vi "TDMS to Patch Image.vi"(0 "Experiment Path":path, 11 "error in (no error)":errorcluster, 12 "Imaging Protocol":T2=enum."Functional Acquisition", 13 "Predominant ROI type":T1=enum."Rectangle", 14 "No of Patches in Experiment":i32) -> (4 "Current Trial Number":i32, 6 "Cancelled":bool, 10 "All Files in Dir":path[](array[path]), 15 "error out":errorcluster)   [LabVIEW 2020]
uses:
  Globals/gl_funct TIFF export globals.vi
  Typedefs/Imaging Protocols enum.ctl
  Typedefs/ROI ID Enum.ctl
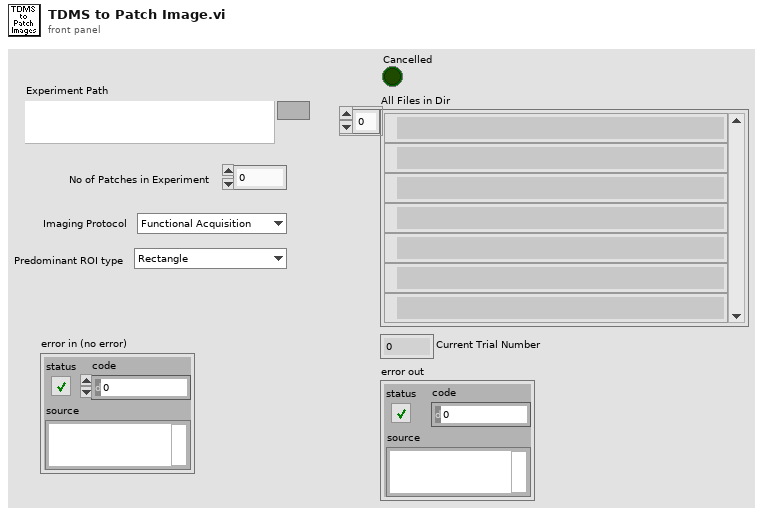
[diagram p1: front panel]
types:
  T1 = typedef "ROI ID Enum.ctl" = enum16{"Point", "MiniScan", "Comp. MiniScan", "Rectangle", "Comp. volume", "Arb. plane point", "None"}
  T2 = typedef "Imaging Protocols enum.ctl" = enum16{"AOL Z-Stack", "Motor Z Stack", "Parameter Sweep", "Functional Acquisition", "Single Plane Acquisition", "Volume Acquisition", "Live Imaging", "Live Plane Imaging", "Live Volume Imaging"}
  T3 = typedef "Funct TIFF exporter ctrl refs.ctl" = cluster{"This VI":refnum<vi>, "Current Experiment":refnum<vi>, "Imaging protocol":refnum<vi>, "Predominant ROI type":refnum<vi>, "Patches in Experiment":refnum<vi>, "Folder Path":refnum<vi>, "Export":refnum<vi>, "Trial number":refnum<vi>, "Output TIFF type":refnum<vi>}
  T4 = typedef "Exported TIFF type.ctl" = enum16{"One multi-page TIFF file for each rectangle", "Individual TIFF files"}
  T5 = typedef "Fixed strings.ctl" = cluster{"ROI file name":string, "Normalised ROI file name":string, "Zplane Pockels values file name":string, "Functional data folder name":string, "Experiment Header file name":string, "Z-stack images folder name":string, "Groups setup rel. path":string, "Groups text file rel. path":string, "TDMS files folder name (F.img)":string, "TDMS files folder name (V.acq)":string, "TDMS files folder name (Pl.acq)":string, "Cycle rel times sequence file":string, "Dynamically called VIs folder name":string, "Time Series folder base name":string, "Parameter Sweep":string}
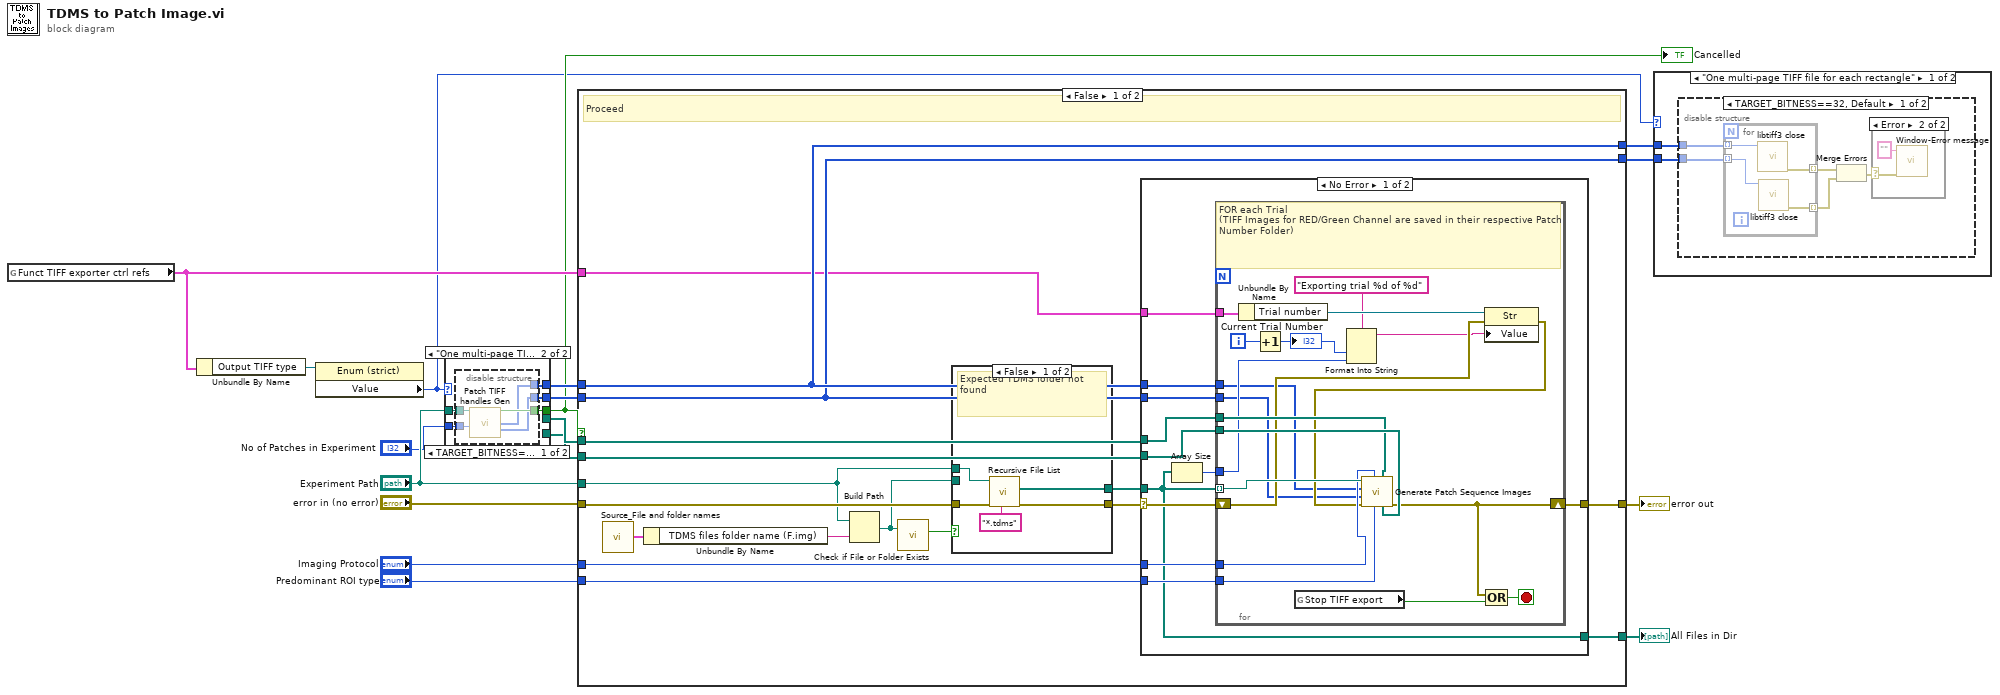
[diagram p0: block diagram]
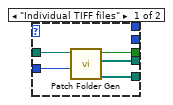
[diagram p5: hidden frame]
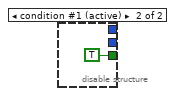
[diagram p6: hidden frame]
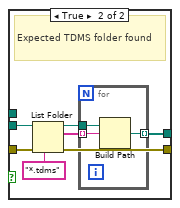
[diagram p7: hidden frame]
diagram:
  n1 = global read "gl_funct TIFF export globals.vi" "Funct TIFF exporter ctrl refs"() -> (w3:T3)
  n2 = Unbundle By Name(w3) -> ("Output TIFF type"=w4:refnum<vi>)
  n3 = property class="Enum (strict)"(reference=w4) -> ("Value"=w1:T4)  [unwired: 1 in, 2 out]
  n4 = case shown="\"One multi-page TIFF file for each rectangle\", Default" w1 {
    tunnel: [w22 _] -> w17
    tunnel: [w21 _] -> w16
    tunnel: [w20 w27] -> w2
    tunnel: "Experiment Path" -> [w19 w26]
    tunnel: "No of Patches in Experiment" -> [w18 w25]
    tunnel: [_ w24] -> w8
    tunnel: [_ w23] -> w7
    frame "Individual TIFF files" {
      n5 = call "Patch Folder Gen.vi"("No of Patches"=w18, "Experimental Folder"=w19) -> ("Green"=w21:path[], "Red"=w22:path[], "Cancelled"=w20:bool)  [unwired: 7 in]
    }
    frame "One multi-page TIFF file for each rectangle", Default {
      n6 = disable-structure shown="TARGET_BITNESS==32, Default" {
        disable-tunnel: [w32 TRUE ("Cancelled")] -> w27
        disable-tunnel: w26 -> [w31 _]
        disable-tunnel: w25 -> [w30 _]
        disable-tunnel: [w29 _] -> w24
        disable-tunnel: [w28 _] -> w23
        frame condition #0 {
          n7 = call "Patch TIFF handles Gen.vi"("Experimental Folder"=w31, "No of Patches"=w30) -> ("Cancelled"=w32:bool, "Red TIFF handles"=w29:i32[], "Green TIFF handles"=w28:i32[])  [unwired: 9 in, 2 out]
        }
        frame condition #1 (active) {
        }
      }
    }
  }
  "Cancelled" <- w2
  n8 = case shown="False" w2 {
    tunnel: w17 -> [w50 _]
    tunnel: w16 -> [w49 _]
    tunnel: "Imaging Protocol" -> [w48 _]
    tunnel: "Predominant ROI type" -> [w47 _]
    tunnel: [w46 w99] -> w12
    tunnel: "error in (no error)" -> [w44 w99]
    tunnel: [w45 _] -> w11
    tunnel: "Experiment Path" -> [w37 _]
    tunnel: w8 -> [w36 w98]
    tunnel: w7 -> [w35 w97]
    tunnel: [w36 w98] -> w6
    tunnel: [w35 w97] -> w5
    tunnel: w3 -> [w34 _]
    frame False {
      # "Proceed"
      n9 = call "Source_File and folder names.vi"() -> ("Fixed strings"=w41:T5)  [unwired: 1 in]
      n10 = Unbundle By Name(w41) -> ("TDMS files folder name (F.img)"=w40:string)
      n11 = Build Path(base path=w37, name or relative path=w40) -> (appended path=w38:path)
      n12 = call <vilib>:"Check if File or Folder Exists.vi"("path"=w38) -> ("file or folder exists?"=w39:bool)  [unwired: 8 in, 2 out]
      n13 = case shown="False" w39 {
        tunnel: w44 -> [w55 w62]
        tunnel: [w54 w61] -> w43
        tunnel: [w53 w56] -> w42
        tunnel: w38 -> [_ w60]
        tunnel: w37 -> [w51 _]
        frame False {
          # "Expected TDMS folder not found"
          n14 = call <vilib>:"Recursive File List.vi"("pattern"="*.tdms", "error in (no error)"=w55, "Folder Path"=w51) -> ("error out"=w54:errorcluster, "All Files in Dir"=w53:path[])  [unwired: 4 in, 3 out]
        }
        frame True {
          # "Expected TDMS folder found"
          n15 = List Folder(path=w60, pattern="*.tdms", error in=w62) -> (path out=w57:path, filenames=w58:string[], error out=w61:errorcluster)  [unwired: 1 in, 1 out]
          n16 = for {
            tunnel: w58 -> [w64] mode=indexing
            tunnel: w57 -> [w65]
            tunnel: [w63] -> w56 mode=indexing
            n17 = Build Path(base path=w65, name or relative path=w64) -> (appended path=w63:path)
          }
        }
      }
      n18 = case shown="No Error" w43 {
        selector: w43 -> [w71 w96]
        tunnel: w42 -> [w69 _]
        tunnel: w50 -> [w76 _]
        tunnel: w49 -> [w75 _]
        tunnel: w48 -> [w74 _]
        tunnel: w47 -> [w73 _]
        tunnel: [w72 w96] -> w46
        tunnel: [w69 _] -> w45
        tunnel: w34 -> [w70 _]
        tunnel: w36 -> [w67 _]
        tunnel: w35 -> [w66 _]
        frame No Error {
          n19 = Array Size(array=w69) -> (size(s)=w68:i32)
          n20 = for {
            tunnel: w69 -> [w95] mode=indexing
            tunnel: w76 -> [w93]
            tunnel: w75 -> [w94]
            tunnel: w74 -> [w92]
            tunnel: w73 -> [w91]
            shift-right: [w88] -> w72
            shift-left: w71 -> [w85]
            tunnel: w70 -> [w87]
            tunnel: w68 -> [w81]
            tunnel: w67 -> [w79]
            tunnel: w66 -> [w78]
            i -> [w77]
            stop <- w89 stop-if-true
            # "FOR each Trial\n(TIFF Images for RED/Green Channel are saved in their respective Patch Number Folder)"
            n21 = Unbundle By Name(w87) -> ("Trial number"=w86:refnum<vi>)
            n22 = Increment(x=w77) -> (x+1=w82:i32)
            "Current Trial Number" <- w82
            n23 = global read "gl_funct TIFF export globals.vi" "Stop TIFF export"() -> (w90:bool)
            n24 = Format Into String(format string="Exporting trial %d of %d", w82, w81) -> (resulting string=w80:string)  [unwired: 2 in, 1 out]
            n25 = property class="Str"(reference=w86, error in=w85, "Value"=w80) -> (error out=w84:errorcluster)  [unwired: 1 out]
            n26 = call "Generate Patch Sequence Images.vi"("Green"=w94, "Red"=w93, "Predominant ROI type"=w91, "Imaging Protocol"=w92, "error in (no error)"=w84, "Green TIFF handles"=w78, "Red TIFF handles"=w79, "TDMS file path & name"=w95) -> ("error out"=w88:errorcluster)  [unwired: 2 in, 1 out]
            n27 = Compound Arithmetic op=OR(w88, w90) -> (w89:bool)
          }
        }
        frame Error {
        }
      }
    }
    frame True {
      # "Error or cancelled"
    }
  }
  "error out" <- w12
  "All Files in Dir" <- w11
  n28 = case shown="\"One multi-page TIFF file for each rectangle\"" w1 {
    tunnel: w6 -> [w101 _]
    tunnel: w5 -> [w100 _]
    frame "One multi-page TIFF file for each rectangle" {
      n29 = disable-structure shown="TARGET_BITNESS==32, Default" {
        disable-tunnel: w101 -> [w106 _]
        disable-tunnel: w100 -> [w105 _]
        frame condition #0 {
          n30 = for {
            tunnel: w106 -> [w112] mode=indexing
            tunnel: w105 -> [w111] mode=indexing
            tunnel: [w110] -> w103 mode=indexing
            tunnel: [w109] -> w104 mode=indexing
            n31 = call "libtiff3 close.vi"("Handle"=w112) -> ("error out"=w109:errorcluster)  [unwired: 9 in]
            n32 = call "libtiff3 close.vi"("Handle"=w111) -> ("error out"=w110:errorcluster)  [unwired: 9 in]
          }
          n33 = Merge Errors(w104, w103) -> (w102:errorcluster)
          n34 = case shown="Error" w102 {
            selector: w102 -> [_ w108]
            frame No Error {
            }
            frame Error {
              n35 = call "Window-Error message.vi"("error in (no error)"=w108, "Message"="") -> ()  [unwired: 9 in, 1 out]
            }
          }
        }
        frame condition #1 (active) {
        }
      }
    }
    frame "Individual TIFF files", Default {
    }
  }
